vi "SubVI_position_sampling_all_bits.vi"(1 "Sample rate":refnum<vi>, 2 "Sampled current position":refnum<vi>, 3 "Decoder main":refnum<vi>, 4 "Bytes at buffer":refnum<vi>, 7 "Stop ALL":refnum<vi>, 8 "Error IN (no error)":errorcluster caption="エラー入力 (エラーなし)", 9 "data bits (8)":u16=8 caption="データビット (8)" min=5 max=8 step=1, 10 "baud rate (115200)":u32=115200 caption="ボーレート (115200)", 11 "VISA resource name":refnum<visa-resource-name>="COM14" caption="VISAリソース名") -> (0 "Error OUT":errorcluster caption="エラー出力")   [LabVIEW 2019]
uses:
  <vilib>/Instr/_visa.llb/VISA Configure Serial Port (Instr).vi
panel:
  out "serial count":i32
  out "communication rate":dbl
  out "value":u8
  out "All Updated?":bool
  out "Decoder":i32[](array[numeric])
  out "Sampled Position":dbl[](array[numeric])
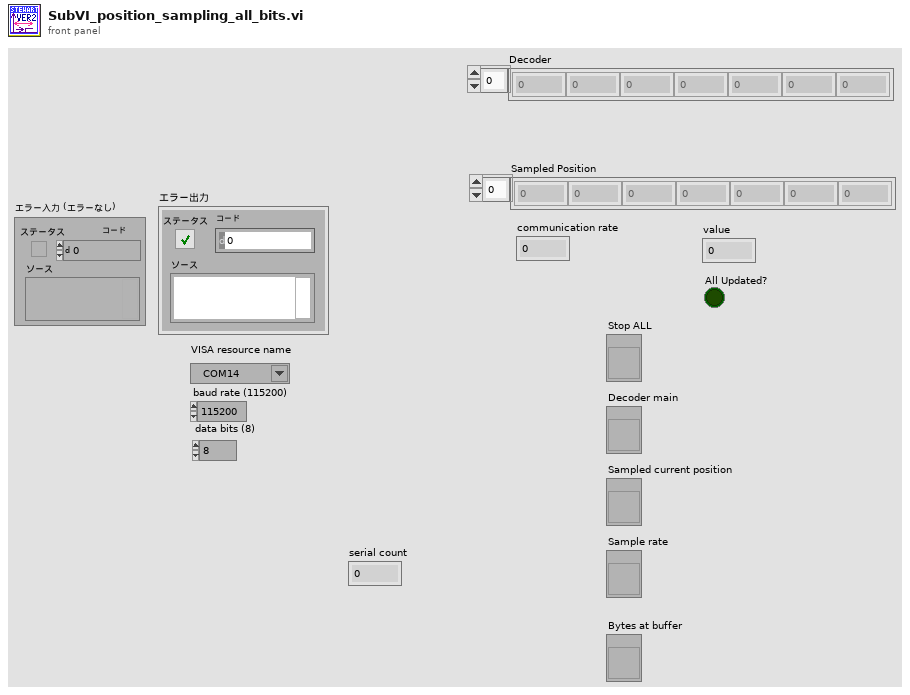
[diagram p1: front panel]
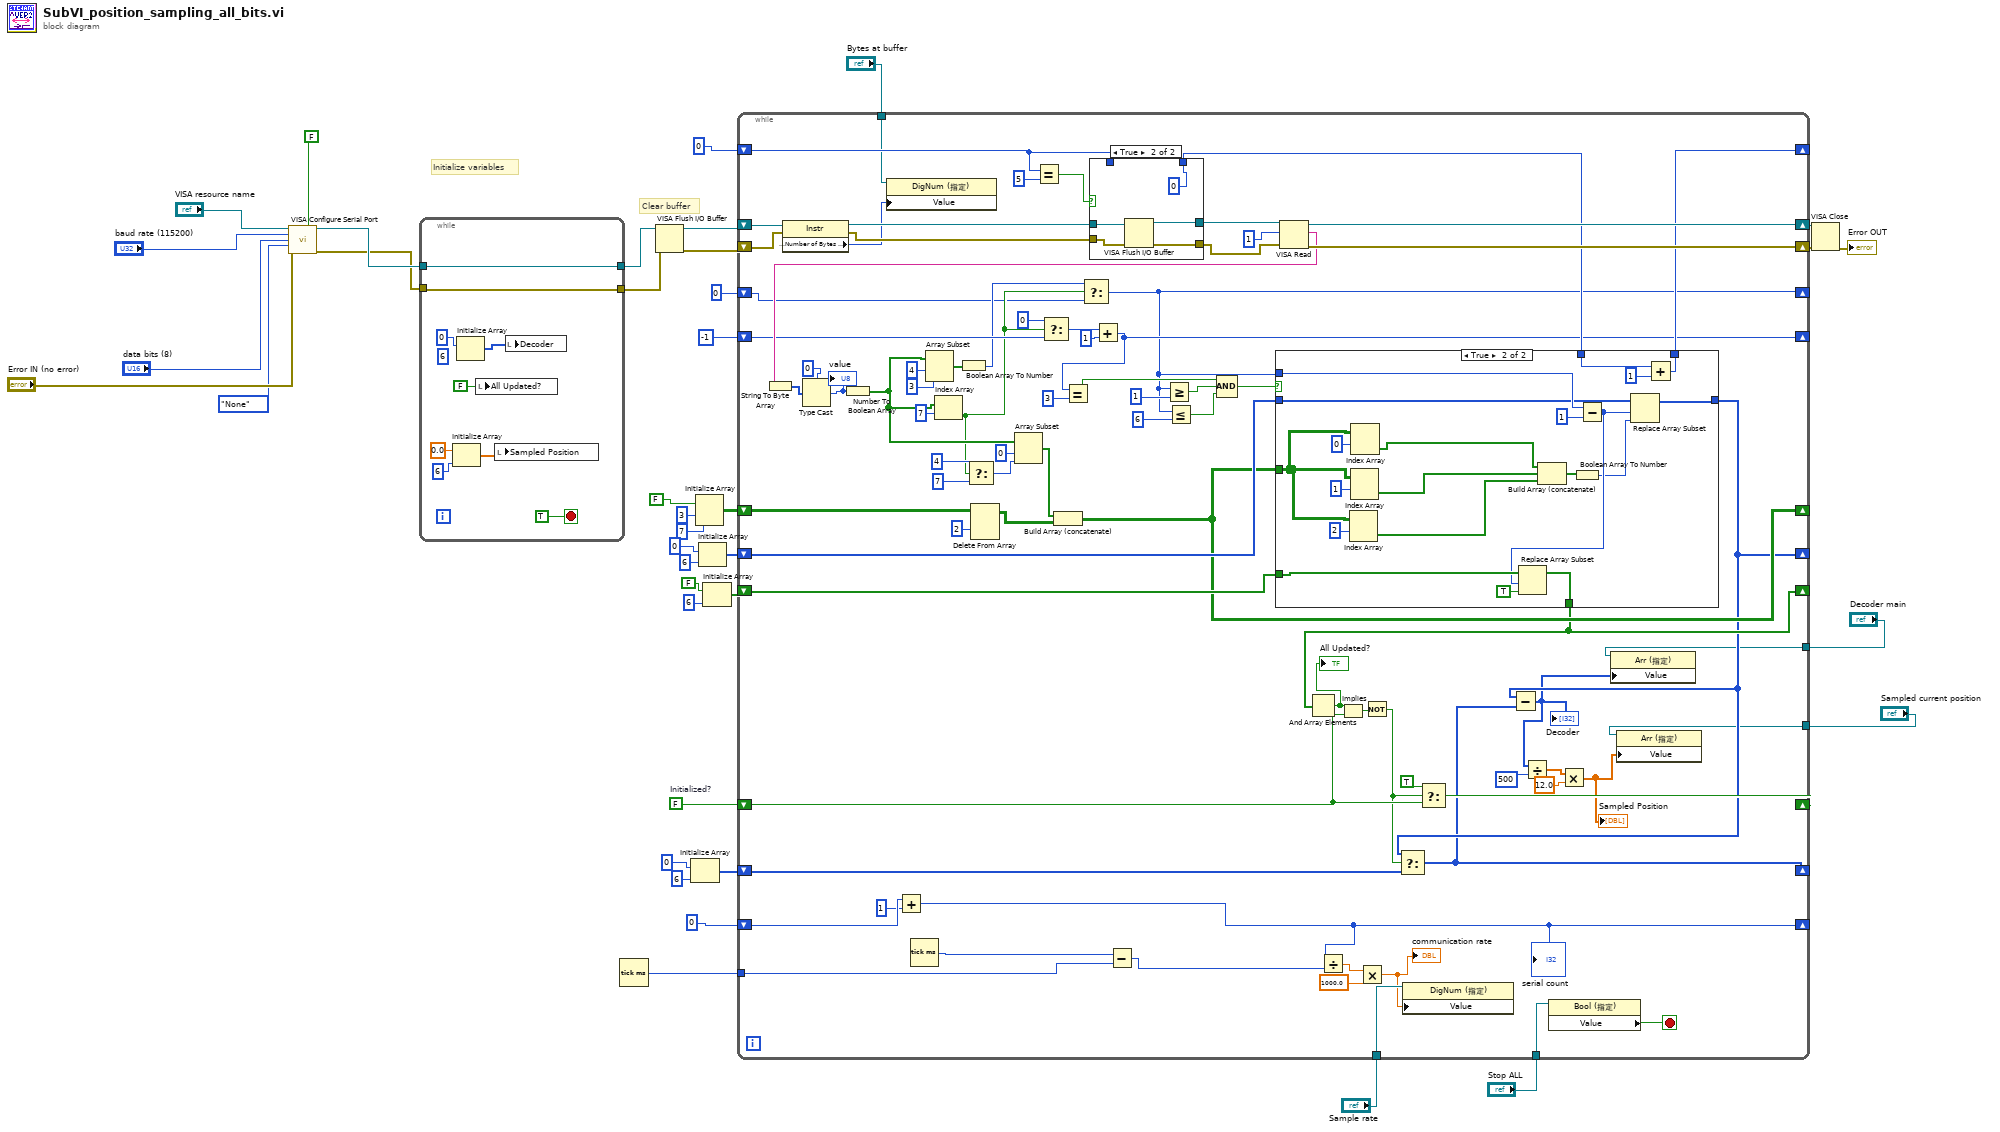
[diagram p0: block diagram]
diagram:
  w12 = FALSE  # Initialized?
  # "Clear buffer"
  # "Initialize variables"
  n1 = call-poly "VISA Configure Serial Port"("VISA resource name"="VISA resource name", "Enable Termination\nChar (T)"=FALSE ("Enable Termination\nChar (T)"), "baud rate (9600)"="baud rate (115200)", "data bits (8)"="data bits (8)", "parity (0:none)"=enum16{"None", "Odd", "Even", "Mark", "Space"}."None", "error in (no error)"="Error IN (no error)") -> ("VISA resource name out"=w11:refnum<visa-resource-name>, "error out"=w10:errorcluster)  [unwired: 8 in]
  n2 = while {
    tunnel: w11 -> [w42]
    tunnel: w10 -> [w41]
    tunnel: [w42] -> w9
    tunnel: [w41] -> w8
    stop <- TRUE stop-if-true
    (unwired) 6 ("次元サイズ")
    n3 = Initialize Array(0.0, 6 ("次元サイズ")) -> (w43:dbl[])
    n4 = Initialize Array(0 ("次元サイズ")) -> (w47:i32[])  [unwired: 1 in]
    n5 = local write "All Updated?"(FALSE ("All Updated?")) -> ()
    n6 = local write "Sampled Position"(w43) -> ()
    n7 = local write "Decoder"(w47) -> ()
  }
  n8 = Tick Count (ms)() -> (millisecond timer value=w20:u32)
  n9 = VISA Flush I/O Buffer(VISA resource name=w9, error in (no error)=w8) -> (VISA resource name out=w22:refnum<visa-resource-name>, error out=w21:errorcluster)  [unwired: 1 in]
  n10 = Initialize Array(0 ("次元サイズ"), 6 ("次元サイズ")) -> (w13:i32[])
  n11 = Initialize Array(FALSE, 3 ("次元サイズ"), 7 ("次元サイズ")) -> (w16:bool[][])
  n12 = Initialize Array(0 ("次元サイズ"), 6 ("次元サイズ")) -> (w32:i32[])
  n13 = Initialize Array(FALSE, 6 ("次元サイズ")) -> (w35:bool[])
  n14 = while {
    shift-right: [w129] -> w31
    shift-left: w22 -> [w110]
    shift-right: [w128] -> w30
    shift-left: w21 -> [w109]
    shift-right: [w111] -> _
    shift-left: 0 -> [w127]
    shift-right: [w92] -> _
    shift-left: w35 -> [w112]
    shift-right: [w84] -> _
    shift-left: w32 -> [w113]
    shift-right: [w108] -> _
    shift-left: u32 0 -> [w103]
    tunnel: w20 -> [w99]
    shift-right: [w93] -> _
    shift-left: w16 -> [w96]
    shift-right: [w83] -> _
    shift-left: w13 -> [w85]
    shift-right: [w87] -> _
    shift-left: w12 -> [w88]
    shift-right: [w70] -> _
    shift-left: -1 -> [w76]
    shift-right: [w59] -> _
    shift-left: u32 0 ("数値") -> [w66]
    tunnel: "Stop ALL" -> [w58]
    tunnel: "Bytes at buffer" -> [w56]
    tunnel: "Sample rate" -> [w54]
    tunnel: "Sampled current position" -> [w52]
    tunnel: "Decoder main" -> [w50]
    stop <- w57 stop-if-true
    n15 = property class="Instr"(reference=w110, error in=w109) -> (reference out=w107:refnum<visa-resource-name>, error out=w106:errorcluster, "Serial Settings:Number of Bytes at Serial Port"=w55:u32)
    n16 = property class="DigNum (指定)"(reference=w56, "Value"=w55) -> ()  [unwired: 1 in, 2 out]
    n17 = Add(x=w127, y=1) -> (x+y=w111:i32)
    "serial count" <- w111
    n18 = Tick Count (ms)() -> (millisecond timer value=w125:u32)
    n19 = Delete From Array(array=w96, index (row)=2 ("指標 (行)")) -> (array with subset deleted=w98:bool[][])  [unwired: 2 in, 1 out]
    n20 = Equal?(x=w103, y=u32 5) -> (x = y?=w104:bool)
    n21 = case shown="TRUE" w104 {
      tunnel: w107 -> [w131 w137]
      tunnel: w106 -> [w130 w136]
      tunnel: [w131 w135] -> w101
      tunnel: [w130 w134] -> w100
      tunnel: w103 -> [w132 _]
      tunnel: [w132 u32 0 ("y")] -> w102
      frame False {
      }
      frame True {
        n22 = VISA Flush I/O Buffer(VISA resource name=w137, error in (no error)=w136) -> (VISA resource name out=w135:refnum<visa-resource-name>, error out=w134:errorcluster)  [unwired: 1 in]
      }
    }
    n23 = Subtract(x=w125, y=w99) -> (x-y=w124:u32)
    n24 = VISA Read(VISA resource name=w101, byte count=u32 1 ("バイトカウント"), error in (no error)=w100) -> (VISA resource name out=w129:refnum<visa-resource-name>, read buffer=w120:string, error out=w128:errorcluster)  [unwired: 1 out]
    n25 = String To Byte Array(string=w120) -> (unsigned byte array=w119:u8[])
    n26 = Type Cast(type=u8 0, x=w119) -> (*(type *) &x=w126:u8)
    "value" <- w126
    n27 = Number To Boolean Array(number=w126) -> (Boolean array=w79:bool[])
    n28 = Array Subset(array=w79, index=4 ("指標"), length=3 ("長さ")) -> (w95:bool[])
    n29 = Index Array(array=w79, index=7 ("指標")) -> (element=w68:bool)
    n30 = Boolean Array To Number(Boolean array=w95) -> (number=w67:u32)
    n31 = Select(t=4 ("長さ"), s=w68, f=7 ("長さ")) -> (s? t:f=w71:i32)
    n32 = Array Subset(array=w79, index=0 ("指標"), length=w71) -> (w94:bool[])
    n33 = Select(t=0, s=w68, f=w76) -> (s? t:f=w75:i32)
    n34 = Build Array (concatenate)(w94, w98) -> (w93:bool[][])
    n35 = Select(t=w67, s=w68, f=w66) -> (s? t:f=w59:u32)
    n36 = Add(x=w75, y=1 ("x")) -> (x+y=w70:i32)
    n37 = Equal?(x=w70, y=3) -> (x = y?=w61:bool)
    n38 = Greater Or Equal?(x=w59, y=u32 1) -> (x >= y?=w63:bool)
    n39 = Less Or Equal?(x=w59, y=u32 6) -> (x <= y?=w62:bool)
    n40 = Compound Arithmetic op=AND ("複合演算")(w61, w63, w62) -> (w60:bool)
    n41 = case shown="TRUE" w60 {
      tunnel: w59 -> [_ w160]
      tunnel: w112 -> [w140 w158]
      tunnel: [w140 w155] -> w92
      tunnel: w113 -> [w139 w154]
      tunnel: [w139 w153] -> w84
      tunnel: w102 -> [w138 w152]
      tunnel: [w138 w150] -> w108
      tunnel: w93 -> [_ w143]
      frame False {
      }
      frame True {
        n42 = Index Array(array=w143, index (row)=2 ("指標 (行)")) -> (element=w141:bool[])  [unwired: 1 in]
        n43 = Index Array(array=w143, index (row)=1 ("指標 (行)")) -> (element=w144:bool[])  [unwired: 1 in]
        n44 = Index Array(array=w143, index (row)=0 ("指標 (行)")) -> (element=w145:bool[])  [unwired: 1 in]
        n45 = Build Array (concatenate)(w145, w144, w141) -> (w146:bool[])
        n46 = Boolean Array To Number ("ブール配列を数値に変換")(Boolean array=w146) -> (number=w142:i16)
        n47 = Subtract(x=w160, y=u32 1) -> (x-y=w157:u32)
        n48 = Replace Array Subset(array=w158, new element=TRUE ("新規要素/部分配列"), index=w157) -> (w155:bool[])
        n49 = Replace Array Subset(array=w154, new element=w142, index=w157) -> (w153:i32[])
        n50 = Add(x=w152, y=u32 1) -> (x+y=w150:u32)
      }
    }
    n51 = And Array Elements(Boolean array=w92) -> (logical AND=w91:bool)
    "All Updated?" <- w91
    n52 = Divide(x=w111, y=w124) -> (x/y=w123:dbl)
    n53 = Implies(1:w88, 2:w91) -> (0:w90:bool)
    n54 = Multiply(x=w123, y=1000.0) -> (x*y=w53:dbl)
    "communication rate" <- w53
    n55 = Not(x=w90) -> (.not. x?=w86:bool)
    n56 = Select(t=w84, s=w86, f=w85) -> (s? t:f=w83:i32[])
    n57 = property class="DigNum (指定)"(reference=w54, "Value"=w53) -> ()  [unwired: 1 in, 2 out]
    n58 = Select(t=TRUE, s=w86, f=w88) -> (s? t:f=w87:bool)
    n59 = Subtract(x=w84, y=w83) -> (x-y=w49:i32[])
    "Decoder" <- w49
    n60 = Divide(x=w49, y=500) -> (x/y=w81:dbl[])
    n61 = property class="Bool (指定)"(reference=w58) -> ("Value"=w57:bool)  [unwired: 1 in, 2 out]
    n62 = Multiply(x=w81, y=12.0) -> (x*y=w51:dbl[])
    "Sampled Position" <- w51
    n63 = property class="Arr (指定)"(reference=w50, "Value"=w49) -> ()  [unwired: 1 in, 2 out]
    n64 = property class="Arr (指定)"(reference=w52, "Value"=w51) -> ()  [unwired: 1 in, 2 out]
  }
  n65 = VISA Close(VISA resource name=w31, error in (no error)=w30) -> (error out=→"Error OUT":errorcluster)
